vi "[ex ce] Partial Derivatives of f(x1,x2).vi"() -> ()   [LabVIEW 2021]
doc: "CE-Math example.\n\n::: CalcExpress Toolkit :::\nCopyright (c) 2000-2026 Konstantin Shifershteyn. All rights reserved."
uses:
  ce exmpl - 2D difference info.ctl
  <vilib>/gmath/NI_Gmath.lvlib
panel:
  in  "number of grid points for both variables":u32=100 min=10 max=500
  in  "derivative":u16(ring) items=["first variable", "second variable"]
  out "max relative difference":T1 {"relative difference, %" format="%#.6g"; "absolute difference" format="%#.6g"}
  out "max absolute difference":T1 {"relative difference, %" format="%#.6g"; "absolute difference" format="%#.6g"}
  out "speed ratio":dbl format="%.3f"
  out "GM ticks":u32 caption="ms"
  out "GM Graph":dbl[][](graph) caption="G Math"
  out "CE ticks":u32 caption="ms"
  out "CE Graph":dbl[][](graph) caption="CalcExpress"
  in  "formula info":T2={"formula"="2*sinc(2*x1)-cos(4*x2+pi(1/2))", "variable 1"="x1", "variable 2"="x2"}
  in  "End":cluster{"x1":dbl, "x2":dbl}={"x1"=3.0, "x2"=3.0} {"x2" format="%.2f"; "x1" format="%.2f"}
  in  "Start":cluster{"x1":dbl, "x2":dbl}={"x1"=-3.0, "x2"=-3.0} {"x2" format="%.2f"; "x1" format="%.2f"}
  # "NOTE    CalcExpress uses (^) operator to perform bitwise-XOR operation but\nnot exponentiation operation. You have to use double-asterisk (**) operator\nto compute an exponent in a CalcExpress expression. For sample, x**y ."
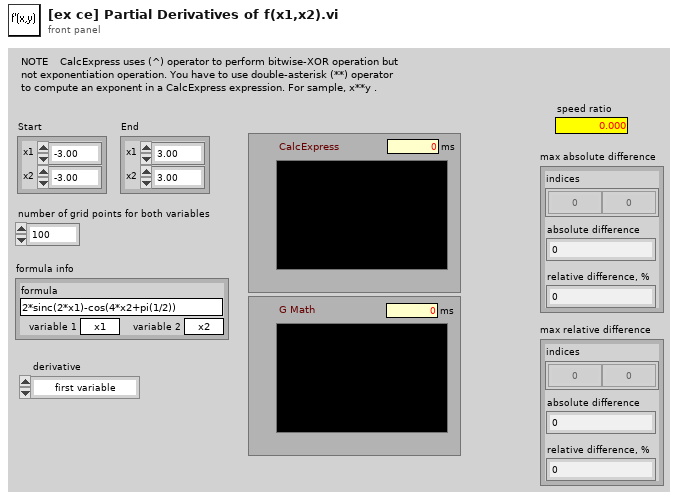
[diagram p1: front panel]
types:
  T1 = typedef "ce exmpl - 2D difference info.ctl" = cluster{"indices":i32[], "absolute difference":dbl, "relative difference, %":dbl}
  T2 = cluster{"formula":string, "variable 1":string, "variable 2":string}
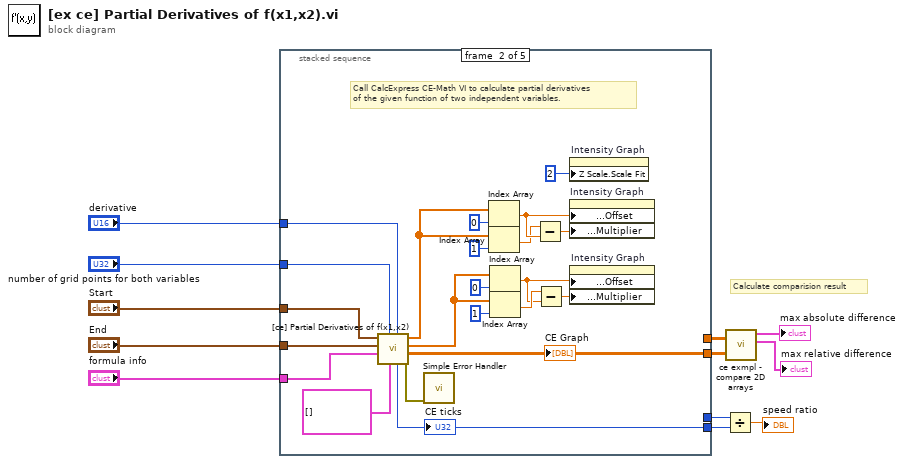
[diagram p0: block diagram]
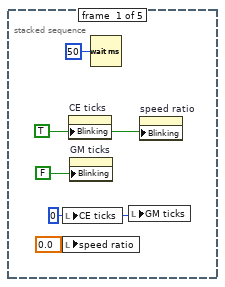
[diagram p2: hidden frame]
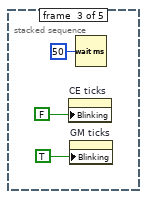
[diagram p3: hidden frame]
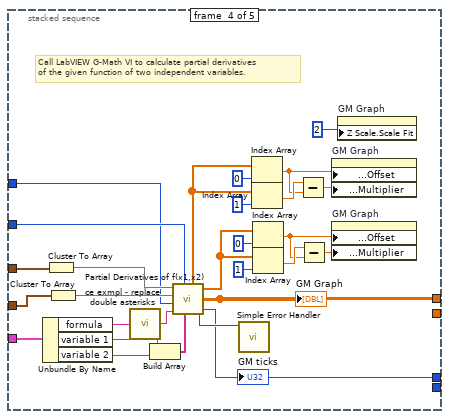
[diagram p4: hidden frame]
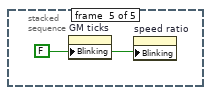
[diagram p5: hidden frame]
diagram:
  # "Calculate comparision result"
  n1 = stacked-sequence {
    tunnel: "Start" -> [_ w24 _ w55 _]
    tunnel: "End" -> [_ w23 _ w54 _]
    tunnel: "formula info" -> [_ w22 _ w53 _]
    tunnel: "number of grid points for both variables" -> [_ w21 _ w56 _]
    tunnel: [_ w18 _ _ _] -> w8
    tunnel: [_ _ _ w52 _] -> w7
    tunnel: [_ w25 _ _ _] -> w6
    tunnel: [_ _ _ w46 _] -> w4
    tunnel: "derivative" -> [_ w20 _ w45 _]
    frame #0 {
      w14 = u32 0 ("CE ticks")
      w16 = TRUE ("Write Attribute")
      n2 = local write "CE ticks"(w14) -> ()
      n3 = local write "speed ratio"(0.0 ("speed ratio")) -> ()
      n4 = property on="CE ticks" class="DigNum (strict)"("Blinking"=w16) -> ()  [unwired: 2 in, 2 out]
      n5 = property on="GM ticks" class="DigNum (strict)"("Blinking"=FALSE ("Write Attribute")) -> ()  [unwired: 2 in, 2 out]
      n6 = Wait (ms)(milliseconds to wait=u32 50) -> ()  [unwired: 1 out]
      n7 = local write "GM ticks"(w14) -> ()
      n8 = property on="speed ratio" class="DigNum (strict)"("Blinking"=w16) -> ()  [unwired: 2 in, 2 out]
    }
    frame #1 {
      # "Call CalcExpress CE-Math VI to calculate partial derivatives\nof the given function of two independent variables."
      n9 = call "[ce] Partial Derivatives of f(x1,x2).vi"("derivative"=w20, "parameters"=cluster{"name":string, "value":dbl}[] [], "# points"=w21, "formula info"=w22, "End"=w23, "Start"=w24) -> ("error out"=w39:errorcluster, "Partial derivative of f(x1,x2)"=w18:dbl[][], "X2  Values"=w29:dbl[], "X1 Values"=w36:dbl[], "ticks"=w25:u32)  [unwired: 1 in]
      "CE Graph" <- w18
      "CE ticks" <- w25
      n10 = call <vilib>:"Simple Error Handler.vi"("error in (no error)"=w39) -> ()  [unwired: 4 in, 5 out]
      n11 = Index Array(array=w36, index=0 ("Index")) -> (element=w38:dbl)
      n12 = Index Array(array=w36, index=1 ("Index")) -> (element=w35:dbl)
      n13 = Index Array(array=w29, index=0 ("Index")) -> (element=w27:dbl)
      n14 = Index Array(array=w29, index=1 ("Index")) -> (element=w30:dbl)
      n15 = Subtract(x=w35, y=w38) -> (x-y=w37:dbl)
      n16 = Subtract(x=w30, y=w27) -> (x-y=w28:dbl)
      n17 = property on="Intensity Graph" class="IntGraph (strict)"("Z Scale.Scale Fit"=u8 2 ("Write Attribute")) -> ()  [unwired: 2 in, 2 out]
      n18 = property on="Intensity Graph" class="IntGraph (strict)"("X Scale.Offset and Multiplier:Offset"=w38, "X Scale.Offset and Multiplier:Multiplier"=w37) -> ()  [unwired: 2 in, 2 out]
      n19 = property on="Intensity Graph" class="IntGraph (strict)"("Y Scale.Offset and Multiplier:Offset"=w27, "Y Scale.Offset and Multiplier:Multiplier"=w28) -> ()  [unwired: 2 in, 2 out]
    }
    frame #2 {
      n20 = property on="CE ticks" class="DigNum (strict)"("Blinking"=FALSE ("Write Attribute")) -> ()  [unwired: 2 in, 2 out]
      n21 = property on="GM ticks" class="DigNum (strict)"("Blinking"=TRUE ("Write Attribute")) -> ()  [unwired: 2 in, 2 out]
      n22 = Wait (ms)(milliseconds to wait=u32 50) -> ()  [unwired: 1 out]
    }
    frame #3 {
      # "Call LabVIEW G-Math VI to calculate partial derivatives\nof the given function of two independent variables."
      n23 = Unbundle By Name(w53) -> ("formula"=w44:string, "variable 1"=w61:string, "variable 2"=w62:string)
      n24 = Cluster To Array(cluster=w55) -> (array=w59:dbl[])
      n25 = Cluster To Array(cluster=w54) -> (array=w60:dbl[])
      n26 = call "ce exmpl - replace double asterisks .vi"("formula in"=w44) -> ("formula out"=w43:string)  [unwired: 4 in]
      n27 = Build Array(w61, w62) -> (w63:string[])
      n28 = call <vilib>:"Partial Derivatives of f(x1,x2).vi"("Variables"=w63, "formula"=w43, "derivative"=w45, "number of points"=w56, "End"=w60, "Start"=w59) -> ("error"=w64:i32, "ticks"=w46:u32, "Partial derivative of f(x1,x2)"=w52:dbl[][], "X2 Values"=w57:dbl[], "X1 Values"=w58:dbl[])
      "GM Graph" <- w52
      "GM ticks" <- w46
      n29 = call <vilib>:"Simple Error Handler.vi"("error code (no error:0)"=w64) -> ()  [unwired: 4 in, 5 out]
      n30 = Index Array(array=w58, index=0 ("Index")) -> (element=w48:dbl)
      n31 = Index Array(array=w58, index=1 ("Index")) -> (element=w70:dbl)
      n32 = Index Array(array=w57, index=0 ("Index")) -> (element=w51:dbl)
      n33 = Index Array(array=w57, index=1 ("Index")) -> (element=w65:dbl)
      n34 = Subtract(x=w70, y=w48) -> (x-y=w49:dbl)
      n35 = Subtract(x=w65, y=w51) -> (x-y=w50:dbl)
      n36 = property on="GM Graph" class="IntGraph (strict)"("X Scale.Offset and Multiplier:Offset"=w48, "X Scale.Offset and Multiplier:Multiplier"=w49) -> ()  [unwired: 2 in, 2 out]
      n37 = property on="GM Graph" class="IntGraph (strict)"("Y Scale.Offset and Multiplier:Offset"=w51, "Y Scale.Offset and Multiplier:Multiplier"=w50) -> ()  [unwired: 2 in, 2 out]
      n38 = property on="GM Graph" class="IntGraph (strict)"("Z Scale.Scale Fit"=u8 2 ("Write Attribute")) -> ()  [unwired: 2 in, 2 out]
    }
    frame #4 {
      w71 = FALSE ("Write Attribute")
      n39 = property on="GM ticks" class="DigNum (strict)"("Blinking"=w71) -> ()  [unwired: 2 in, 2 out]
      n40 = property on="speed ratio" class="DigNum (strict)"("Blinking"=w71) -> ()  [unwired: 2 in, 2 out]
    }
  }
  n41 = Divide(x=w4, y=w6) -> (x/y=→"speed ratio":dbl)
  n42 = call "ce exmpl - compare 2D arrays.vi"("array for checking"=w8, "standard array"=w7) -> ("max relative difference"=→"max relative difference":T1, "max absolute difference"=→"max absolute difference":T1)  [unwired: 1 in, 2 out]
